vi "RFH-read-common_format.vi"(7 "file path (dialog if empty)":path, 8 "error in":errorcluster) -> (0 "error out":errorcluster, 2 "Common Format":T1)   [LabVIEW 2020, in "RFH-Reflection_File_Handler.lvlib"]
doc: "Reads a common-format file (dialog if the path is empty) into a Common Format cluster."
uses:
  RFH-Reflection_File_Handler.lvlib
  RFH-common_data_format.ctl
panel:
  out "Waveform Graph 3":dbl[](graph)
  out "Waveform Graph 2":dbl[](graph)
  out "Waveform Graph":dbl[](graph)
  out "string array 2":string[][](array[string])
  out "string array":string[](array[string])
  out "after substring":string
  out "text":string
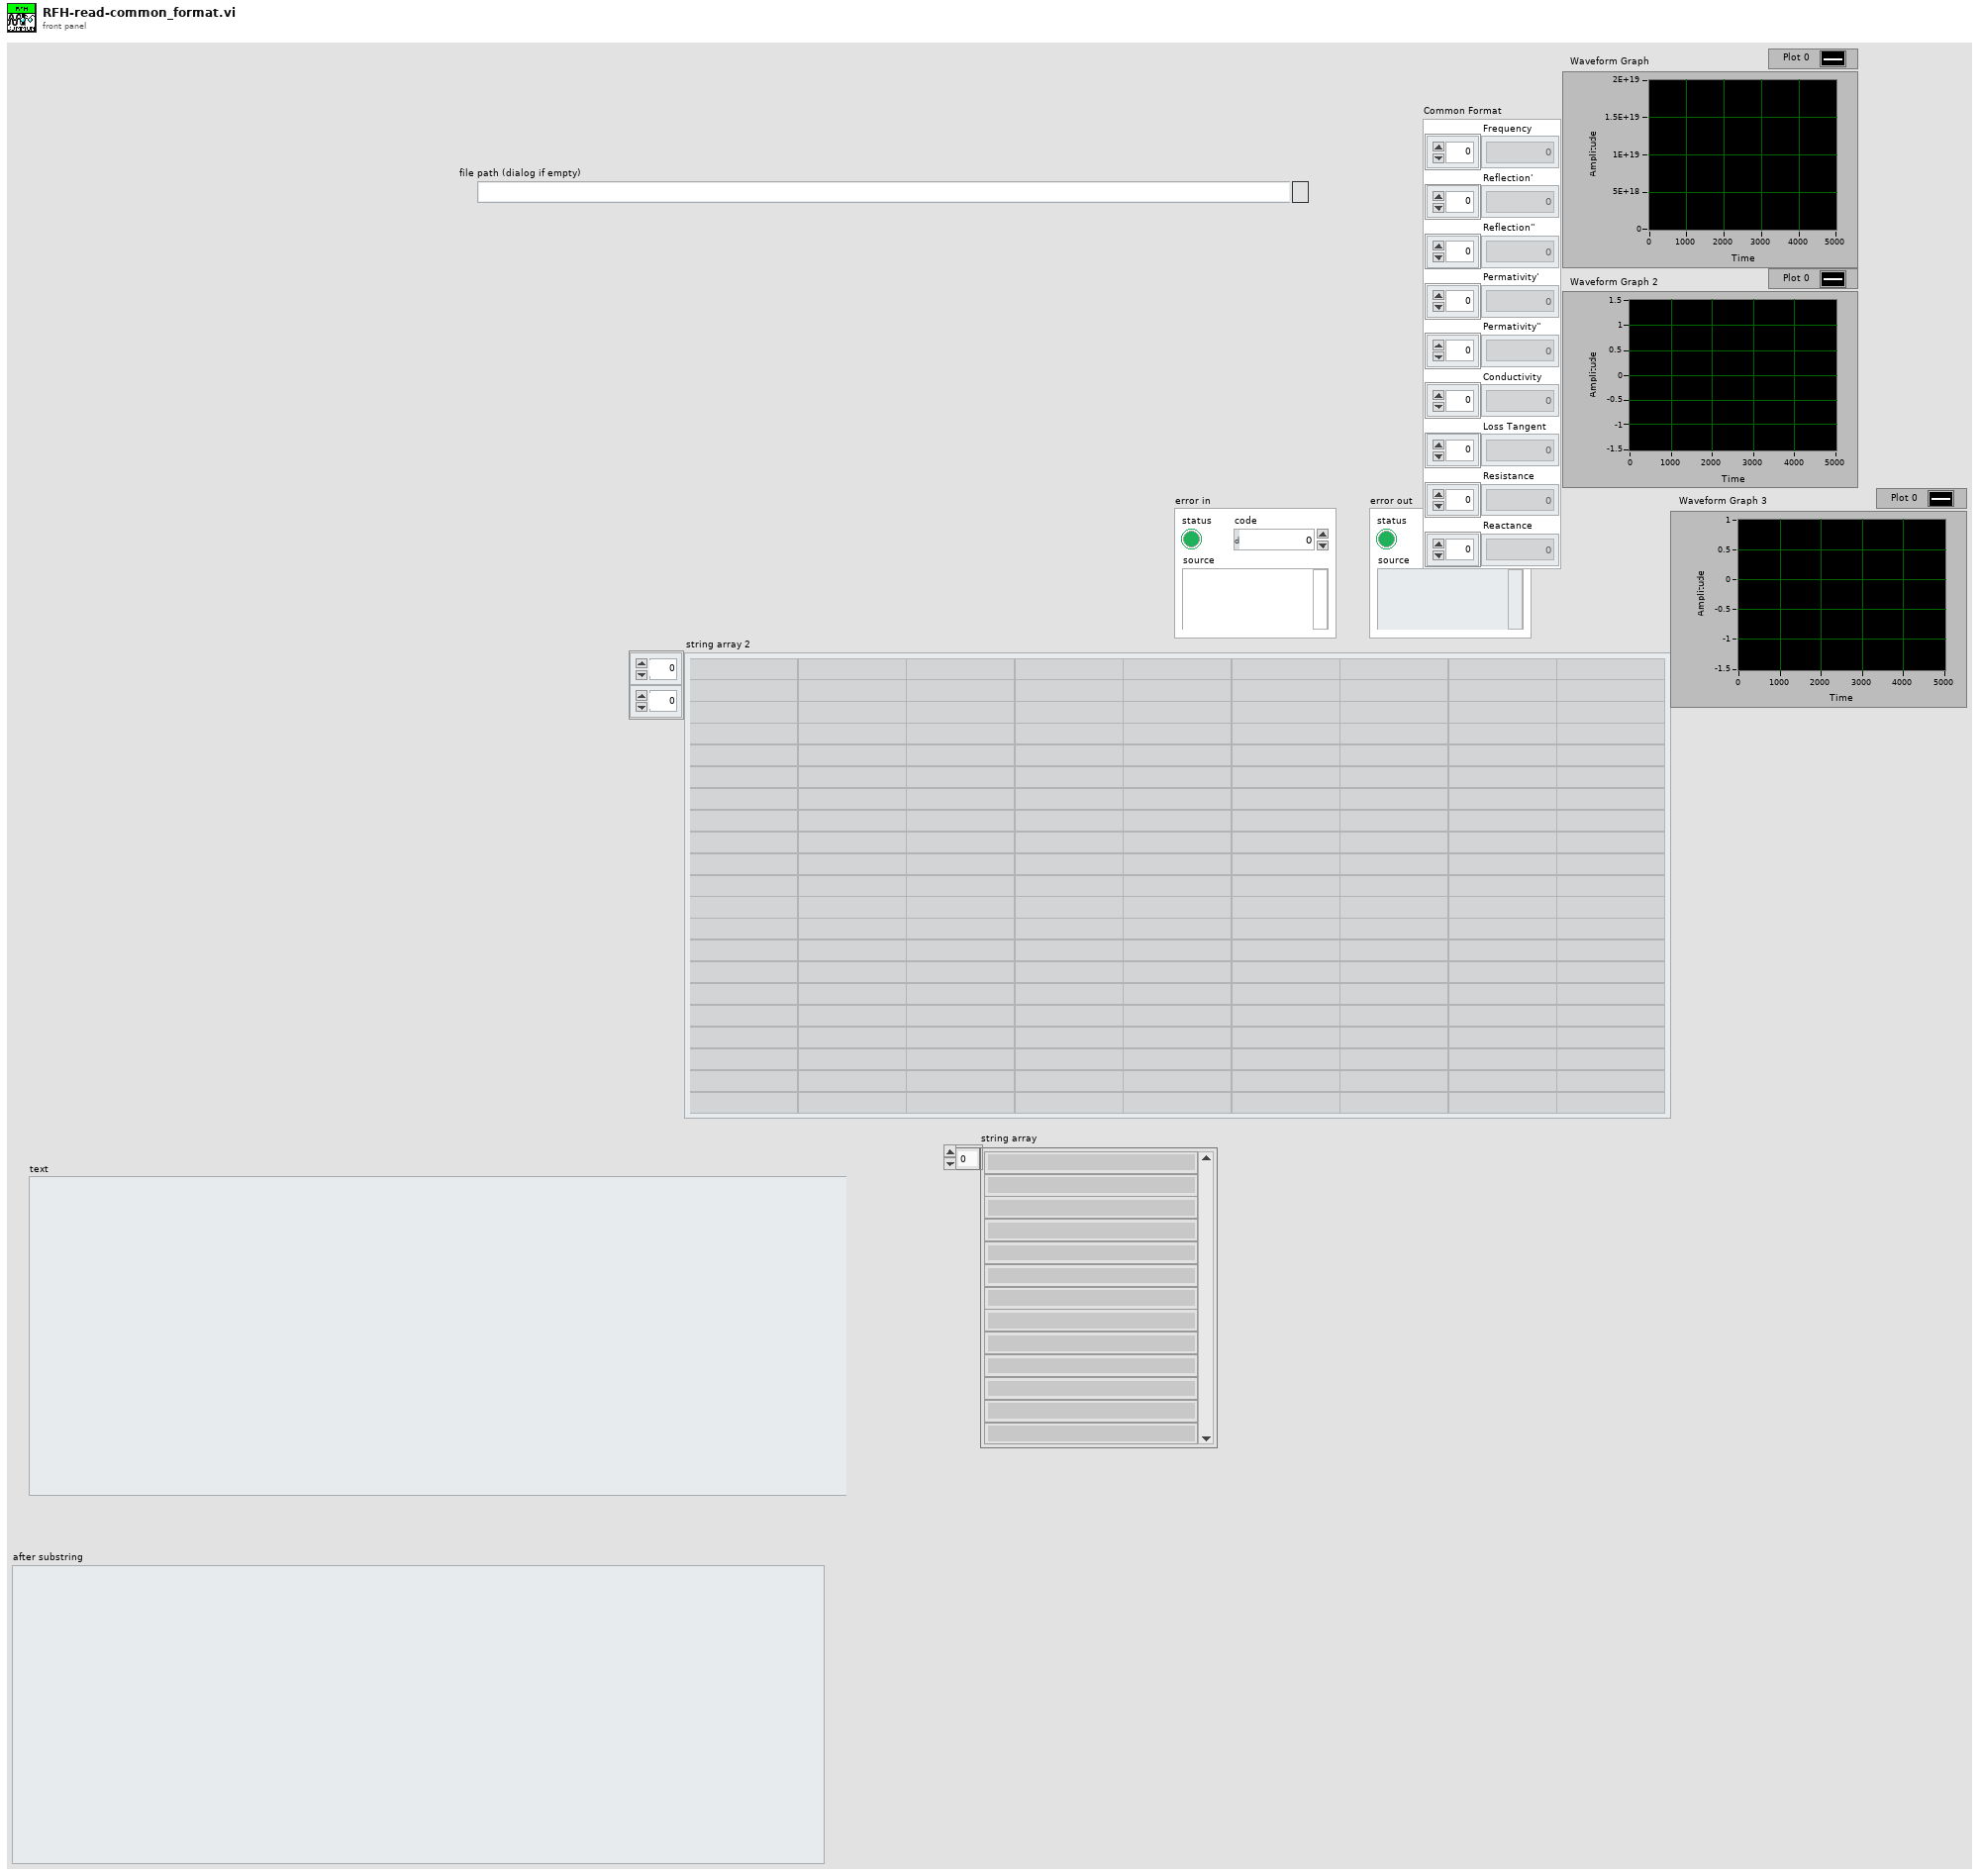
[diagram p1: front panel]
types:
  T1 = typedef "RFH-Reflection_File_Handler.lvlib/RFH-common_data_format.ctl" = cluster{"Frequency":dbl[], "Reflection'":dbl[], "Reflection''":dbl[], "Permativity'":dbl[], "Permativity''":dbl[], "Conductivity":dbl[], "Loss Tangent":dbl[], "Resistance":dbl[], "Reactance":dbl[]}
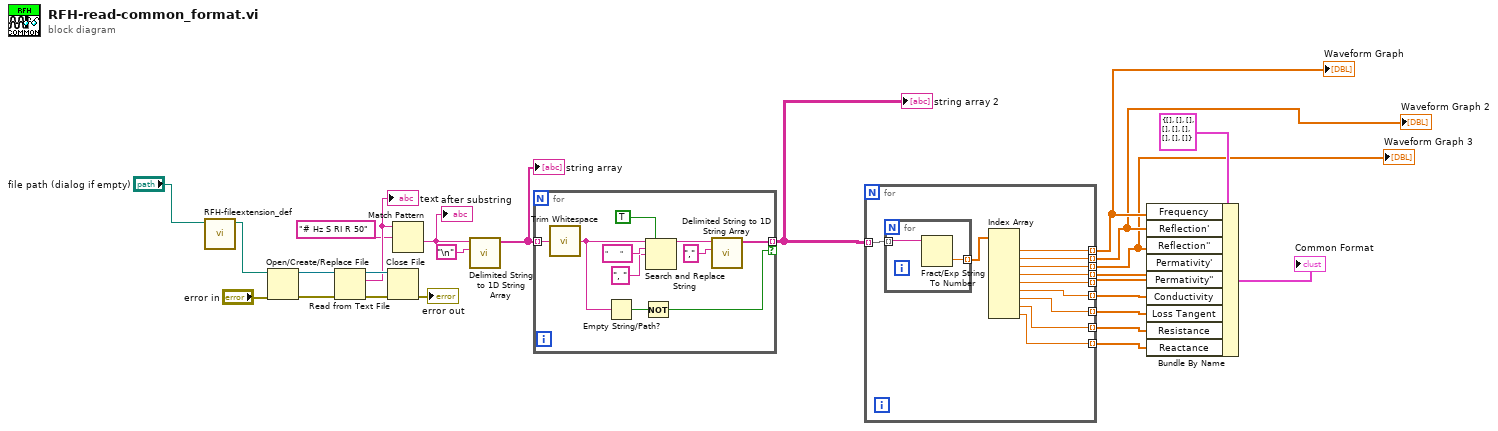
[diagram p0: block diagram]
diagram:
  n1 = call "RFH-fileextension_def.vi"("Path in"="file path (dialog if empty)") -> ("Path with file extention"=w8:path)  [unwired: 9 in, 1 out]
  n2 = Open/Create/Replace File(file path (use dialog)=w8, error in="error in") -> (refnum out=w25:refnum<file>, error out=w22:errorcluster)  [unwired: 4 in, 1 out]
  n3 = Read from Text File(file (use dialog)=w25, error in=w22) -> (refnum out=w24:refnum<file>, text=w21:string, error out=w23:errorcluster)  [unwired: 2 in, 1 out]
  "text" <- w21
  n4 = Close File(refnum=w24, error in=w23) -> (error out=→"error out":errorcluster)  [unwired: 1 out]
  n5 = Match Pattern(string=w21, regular expression="# Hz S RI R 50" ("search string/char (-)")) -> (after substring=w17:string)  [unwired: 1 in, 3 out]
  "after substring" <- w17
  n6 = call <vilib>:"Delimited String to 1D String Array.vi"("delimiter"="\n", "delimited string"=w17) -> ("string array"=w18:string[])  [unwired: 9 in]
  "string array" <- w18
  n7 = for {
    tunnel: w18 -> [w35] mode=indexing
    tunnel: [w34] -> w16 mode=indexing if=w26
    n8 = call <vilib>:"Trim Whitespace.vi"("string"=w35) -> ("trimmed string"=w28:string)  [unwired: 1 in]
    n9 = Empty String/Path?(string/path=w28) -> (empty?=w27:bool)
    n10 = Not(x=w27) -> (.not. x?=w26:bool)
    n11 = Search and Replace String(replace all?=TRUE ("replace all? (F)"), input string=w28, search string="      ", replace string=", " ("replace string (\"\")")) -> (result string=w29:string)  [unwired: 4 in, 3 out]
    n12 = call <vilib>:"Delimited String to 1D String Array.vi"("delimiter"=",", "delimited string"=w29) -> ("string array"=w34:string[])  [unwired: 9 in]
  }
  "string array 2" <- w16
  n13 = for {
    tunnel: w16 -> [w46] mode=indexing
    tunnel: [w44] -> w3 mode=indexing
    tunnel: [w43] -> w2 mode=indexing
    tunnel: [w42] -> w1 mode=indexing
    tunnel: [w41] -> w15 mode=indexing
    tunnel: [w40] -> w14 mode=indexing
    tunnel: [w39] -> w7 mode=indexing
    tunnel: [w38] -> w6 mode=indexing
    tunnel: [w37] -> w5 mode=indexing
    tunnel: [w36] -> w4 mode=indexing
    n14 = for {
      tunnel: w46 -> [w48] mode=indexing
      tunnel: [w47] -> w45 mode=indexing
      n15 = Fract/Exp String To Number(string=w48) -> (number=w47:dbl)  [unwired: 3 in, 1 out]
    }
    n16 = Index Array(array=w45) -> (element #1=w44:dbl, element #2=w43:dbl, element #3=w42:dbl, element #4=w41:dbl, element #5=w40:dbl, element #6=w39:dbl, element #7=w38:dbl, element #8=w37:dbl, element #9=w36:dbl)  [unwired: 9 in]
  }
  "Waveform Graph" <- w3
  "Waveform Graph 2" <- w2
  "Waveform Graph 3" <- w1
  n17 = Bundle By Name(cluster=T1 {"Frequency"=[], "Reflection'"=[], "Reflection''"=[], "Permativity'"=[], "Permativity''"=[], "Conductivity"=[], "Loss Tangent"=[], "Resistance"=[], "Reactance"=[]} ("Common Format"), "Frequency"=w3, "Reflection'"=w2, "Reflection''"=w1, "Permativity'"=w15, "Permativity''"=w14, "Conductivity"=w7, "Loss Tangent"=w6, "Resistance"=w5, "Reactance"=w4) -> (→"Common Format":T1)
